vi "Get T1Data.vi"(8 "error in (no error)":errorcluster caption="错误输入（无错误）", 9 "data":u64[](array[numeric]), 10 "nChannel":i32, 11 "nBoard":i32) -> (0 "error out":errorcluster caption="错误输出", 2 "data 2":u64[](array[numeric]), 3 "function return":i32)   [LabVIEW 2017, in "smncsftmt.lvlib"]
doc: "__declspec(dllexport) int GetT1Data(int nBoard, int nChannel, unsigned long long* data);"
uses:
  smncsftmt.lvlib
  smncsftmt.dll
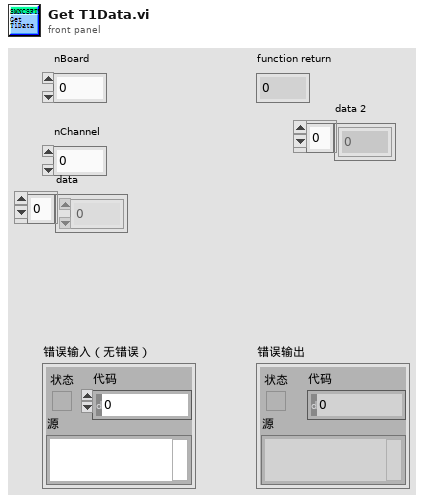
[diagram p1: front panel]
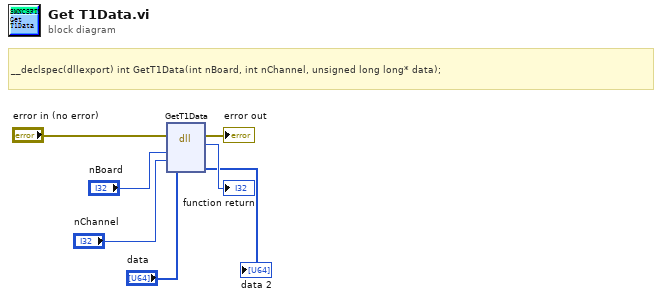
[diagram p0: block diagram]
diagram:
  # "__declspec(dllexport) int GetT1Data(int nBoard, int nChannel, unsigned long long* data);"
  n1 = dll-call lib="PTH2oabs CUsersaDesktop\nLABVIEW范例National InstrumentsLabVIEW 2017user.lib\tsmncsftmtsmncsftmt.*" fn="GetT1Data"(error in="error in (no error)", "nBoard"="nBoard", "nChannel"="nChannel", "data"="data") -> (error out=→"error out":errorcluster, "返回类型"=→"function return":i32, "data"=→"data 2":u64[])  [unwired: 4 in, 1 out]
